vi "Trapezoid Profile Generator.vi"(8 "Starting Position":dbl, 9 "Distance":dbl, 10 "Velocity Max":dbl, 11 "Acceleration Max":dbl) -> (1 "Positions":dbl[](array[numeric]), 2 "Velocity values":dbl[](array[numeric]), 3 "Timestamp":dbl[](array[numeric]) format="%.2f")   [LabVIEW 2027]
panel:
  out "area":sgl
  out "Time":sgl
  out "XY Graph":cluster{dbl[], dbl[]}(graph)
  out "Slope Change Point (seconds)":dbl
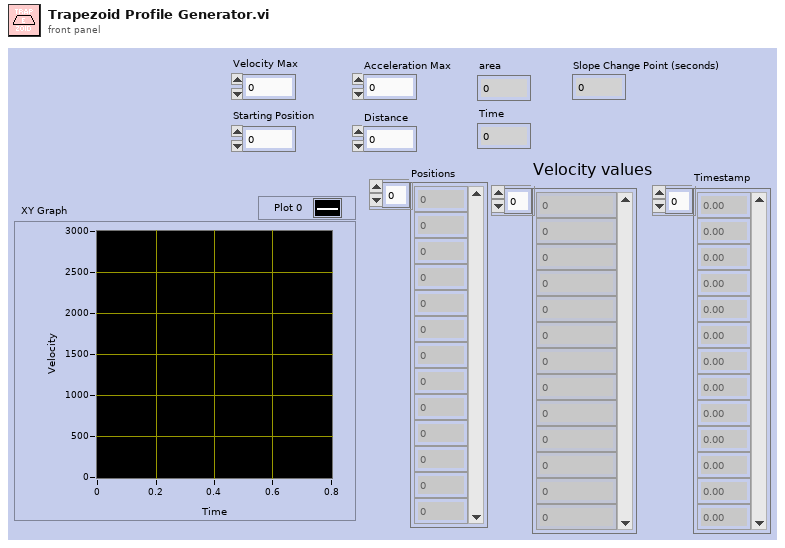
[diagram p1: front panel]
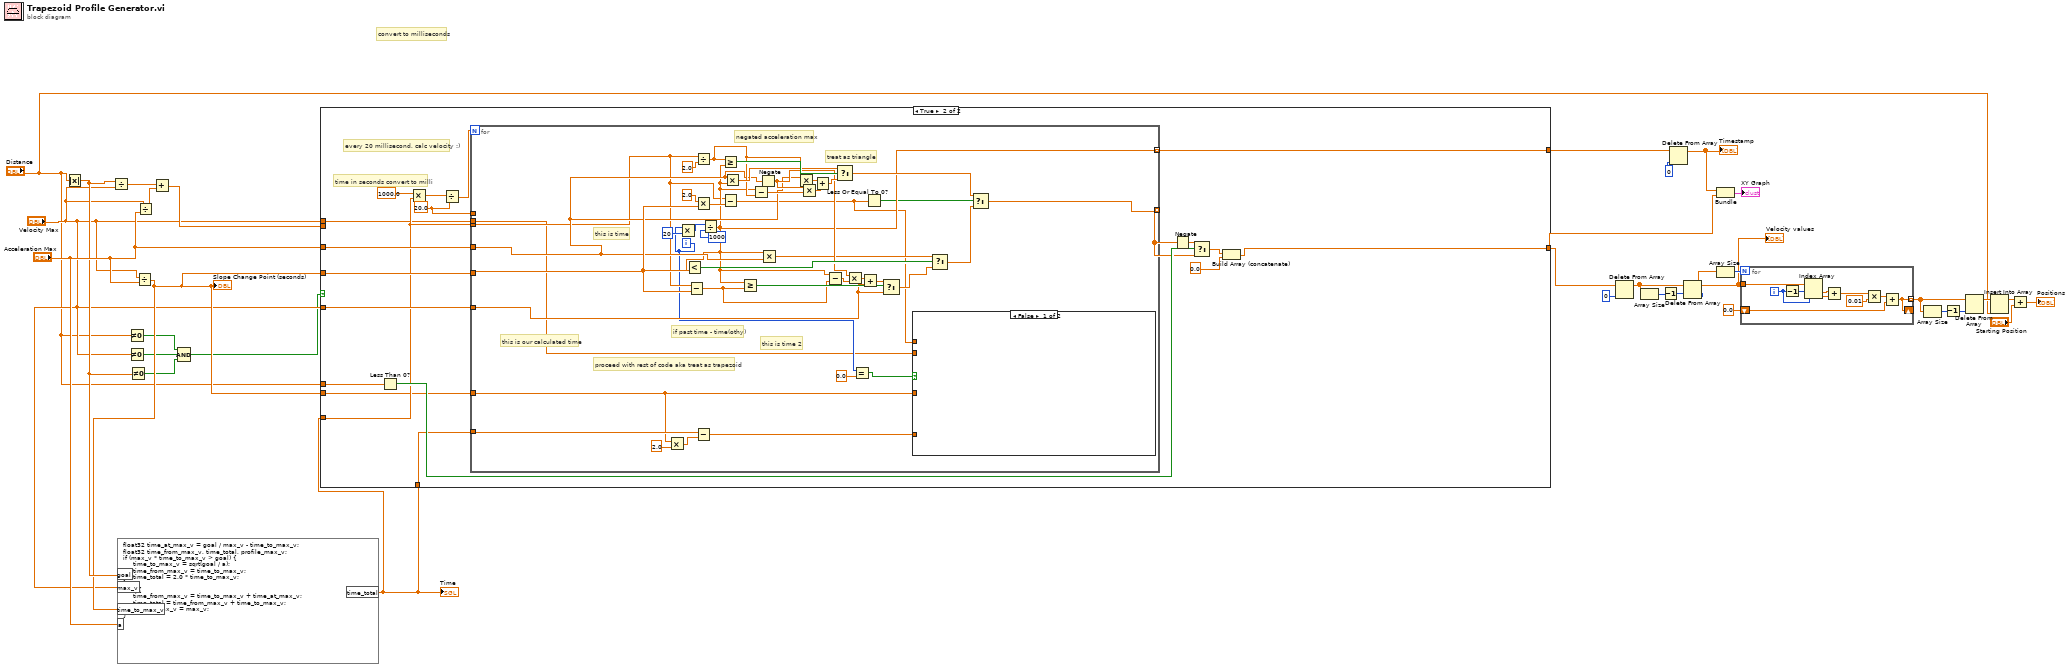
[diagram p0: block diagram]
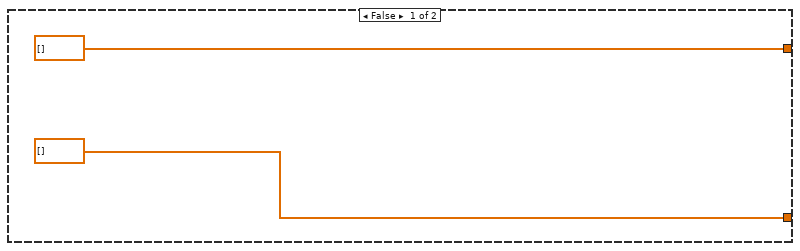
[diagram p2: hidden frame]
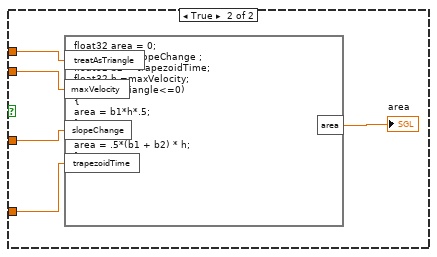
[diagram p3: hidden frame]
diagram:
  # "convert to milliseconds"
  n1 = Absolute Value(x="Distance") -> (abs(x)=w28:dbl)
  n2 = Divide(x=w28, y="Velocity Max") -> (x/y=w30:dbl)
  n3 = Not Equal To 0?(x="Distance") -> (x != 0?=w23:bool)
  n4 = Not Equal To 0?(x="Velocity Max") -> (x != 0?=w24:bool)
  n5 = Not Equal To 0?(x=w28) -> (x != 0?=w25:bool)
  n6 = Divide(x="Velocity Max", y="Acceleration Max") -> (x/y=w27:dbl)
  "Slope Change Point (seconds)" <- w27
  n7 = formula code="float32 time_at_max_v = goal / max_v - time_to_max_v;\nfloat32 time_from_max_v, time_total, profile_max_v;\nif (max_v * time_to_max_v > goal) {\n     time_to_max_v = sqrt(goal / a);\n     time_from_max_v = time_to_max_v;\n     time_total = 2.0 * time_to_max_v;\n}\nelse {\n     time_from_max_v = time_to_max_v + time_at_max_v;\n     time_total = time_from_max_v + time_to_max_v;\n     profile_max_v = max_v;\n}"("goal"=w28, "max_v"="Velocity Max", "time_to_max_v"=w27, "a"="Acceleration Max") -> ("time_total"=w19:sgl)
  "Time" <- w19
  n8 = Divide(x="Velocity Max", y="Acceleration Max") -> (x/y=w32:dbl)
  n9 = Add(x=w30, y=w32) -> (x+y=w31:dbl)
  n10 = Compound Arithmetic op=AND(w23, w24, w25) -> (w22:bool)
  n11 = case shown="True" w22 {
    tunnel: "Velocity Max" -> [_ w53]
    tunnel: w27 -> [_ w52]
    tunnel: [dbl[] [] w39] -> w8
    tunnel: w31 -> [_ _]
    tunnel: "Acceleration Max" -> [_ w50]
    tunnel: [dbl[] [] w40] -> w13
    tunnel: w19 -> [_ w38]
    tunnel: "Distance" -> [_ w45]
    tunnel: "Velocity Max" -> [_ w37]
    tunnel: w27 -> [_ w36]
    tunnel: w19 -> [_ w35]
    frame False {
    }
    frame True {
      w46 = 20.0 ("y")
      # "every 20 millisecond, calc velocity :)"
      # "time in seconds convert to milli"
      n12 = Less Than 0?(x=w45) -> (x < 0?=w48:bool)
      n13 = Multiply(x=1000.0, y=w38) -> (x*y=w51:dbl)
      n14 = Divide(x=w51, y=w46) -> (x/y=w43:dbl)
      n15 = for {
        N: w43 -> [_]
        tunnel: [w86] -> w47 mode=indexing
        tunnel: w50 -> [w76]
        tunnel: w53 -> [w68]
        tunnel: w52 -> [w85]
        tunnel: [w67] -> w39 mode=indexing
        tunnel: w46 -> [_]
        tunnel: w38 -> [w66]
        tunnel: w37 -> [w59]
        tunnel: w36 -> [w55]
        tunnel: w35 -> [w58]
        i -> [w61]
        # "this is our calculated time"
        # "this is time 2"
        # "this is time"
        # "negated acceleration max"
        # "if past time - time(othy)"
        # "treat as triangle"
        # "proceed with rest of code aka treat as trapezoid"
        n16 = Multiply(x=w55, y=2.0) -> (x*y=w57:dbl)
        n17 = Multiply(x=w61, y=20) -> (x*y=w73:i32)
        n18 = Subtract(x=w66, y=w85) -> (x-y=w74:dbl)
        n19 = Divide(x=w66, y=2.0) -> (x/y=w79:dbl)
        n20 = Multiply(x=2.0, y=w85) -> (x*y=w93:dbl)
        n21 = Subtract(x=w58, y=w57) -> (x-y=w54:dbl)
        n22 = Divide(x=w73, y=1000) -> (x/y=w67:dbl)
        n23 = Less?(x=w67, y=w85) -> (x < y?=w87:bool)
        n24 = Greater Or Equal?(x=w79, y=w67) -> (x >= y?=w91:bool)
        n25 = Subtract(x=w66, y=w93) -> (x-y=w60:dbl)
        n26 = Multiply(x=w76, y=w67) -> (x*y=w84:dbl)
        n27 = Greater Or Equal?(x=w67, y=w74) -> (x >= y?=w90:bool)
        n28 = Subtract(x=w67, y=w79) -> (x-y=w83:dbl)
        n29 = Negate(x=w76) -> (-x=w78:dbl)
        n30 = Multiply(x=w67, y=w76) -> (x*y=w71:dbl)
        n31 = Multiply(x=w76, y=w79) -> (x*y=w81:dbl)
        n32 = Multiply(x=w78, y=w83) -> (x*y=w82:dbl)
        n33 = Add(x=w81, y=w82) -> (x+y=w80:dbl)
        n34 = Subtract(x=w67, y=w74) -> (x-y=w69:dbl)
        n35 = Select(t=w84, s=w91, f=w80) -> (s? t:f=w75:dbl)
        n36 = Multiply(x=w78, y=w69) -> (x*y=w77:dbl)
        n37 = Equal?(x=w61, y=0.0) -> (x = y?=w63:bool)
        n38 = Add(x=w77, y=w68) -> (x+y=w70:dbl)
        n39 = Less Or Equal To 0?(x=w60) -> (x <= 0?=w64:bool)
        n40 = Select(t=w70, s=w90, f=w68) -> (s? t:f=w89:dbl)
        n41 = case shown="False" w63 {
          tunnel: w60 -> [_ w99]
          tunnel: w59 -> [_ w97]
          tunnel: w55 -> [_ w96]
          tunnel: w54 -> [_ w95]
          frame False {
          }
          frame True {
            n42 = formula code="float32 area = 0;\nfloat32 b1 =slopeChange ;\nfloat32 b2 = trapezoidTime;\nfloat32 h =maxVelocity; \nif(treatAsTriangle<=0)\n{\narea = b1*h*.5;\n}\nelse{\narea = .5*(b1 + b2) * h;\n}"("treatAsTriangle"=w99, "maxVelocity"=w97, "slopeChange"=w96, "trapezoidTime"=w95) -> ("area"=→"area":sgl)
          }
        }
        n43 = Select(t=w71, s=w87, f=w89) -> (s? t:f=w88:dbl)
        n44 = Select(t=w75, s=w64, f=w88) -> (s? t:f=w86:dbl)
      }
      n45 = Negate(x=w47) -> (-x=w49:dbl[])
      n46 = Select(t=w49, s=w48, f=w47) -> (s? t:f=w42:dbl[])
      n47 = Build Array (concatenate)(w42, 0.0) -> (w40:dbl[])
    }
  }
  n48 = Delete From Array(array=w13, index=0) -> (array with subset deleted=w5:dbl[])  [unwired: 1 in, 1 out]
  n49 = Array Size(array=w5) -> (size(s)=w6:i32)
  n50 = Decrement(x=w6) -> (x-1=w4:i32)
  n51 = Delete From Array(array=w8, index=0) -> (array with subset deleted=w12:dbl[])  [unwired: 1 in, 1 out]
  "Timestamp" <- w12
  n52 = Delete From Array(array=w5, index=w4) -> (array with subset deleted=w7:dbl[])  [unwired: 1 in, 1 out]
  "Velocity values" <- w7
  n53 = Array Size(array=w7) -> (size(s)=w20:i32)
  n54 = Bundle(w12, w13) -> (→"XY Graph":cluster{dbl[], dbl[]})  [unwired: 1 in]
  n55 = for {
    N: w20 -> [_]
    tunnel: w7 -> [w109]
    shift-right: [w102] -> _
    shift-left: 0.0 -> [w108]
    tunnel: [w102] -> w16 mode=indexing
    i -> [w100]
    n56 = Decrement(x=w100) -> (x-1=w101:i32)
    n57 = Index Array(array=w109, index #1=w101, index #2=w100) -> (element #1=w106:dbl, element #2=w107:dbl)
    n58 = Add(x=w106, y=w107) -> (x+y=w105:dbl)
    n59 = Multiply(x=w105, y=0.01) -> (x*y=w103:dbl)
    n60 = Add(x=w103, y=w108) -> (x+y=w102:dbl)
  }
  n61 = Array Size(array=w16) -> (size(s)=w18:i32)
  n62 = Decrement(x=w18) -> (x-1=w17:i32)
  n63 = Delete From Array(array=w16, index=w17) -> (array with subset deleted=w10:dbl[])  [unwired: 1 in, 1 out]
  n64 = Insert Into Array(array=w10, new element="Distance") -> (w3:dbl[])  [unwired: 1 in]
  n65 = Add(x=w3, y="Starting Position") -> (x+y=→"Positions":dbl[])
